vi "set Reference Level.vi"(8 "error in (no error)":errorcluster, 10 "Reference Level":dbl, 11 "Keysight 9020A in":refnum<class "Keysight 9020A.lvclass">) -> (0 "error out":errorcluster, 3 "Keysight 9020A out":refnum<class "Keysight 9020A.lvclass">)   [LabVIEW 2023, in "Spectrum Analyzer.lvlib" / "Keysight 9020A.lvclass"]
uses:
  Keysight 9020A.lvclass
  Keysight 9020A.lvclass/Keysight 9020A.ctl
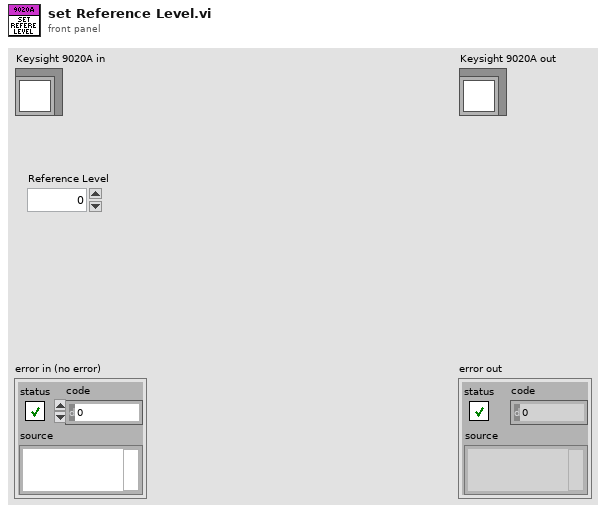
[diagram p1: front panel]
types:
  T1 = typedef "Spectrum Analyzer.lvlib/TYPE Measurement Preset.ctl" = enum16{"Sweep SA Mode", "Channel Power", "Occupied BW", "ACP", "Spurious Emission", "Spurious Emission Mask", "Burst Power (Transmit Power)"}
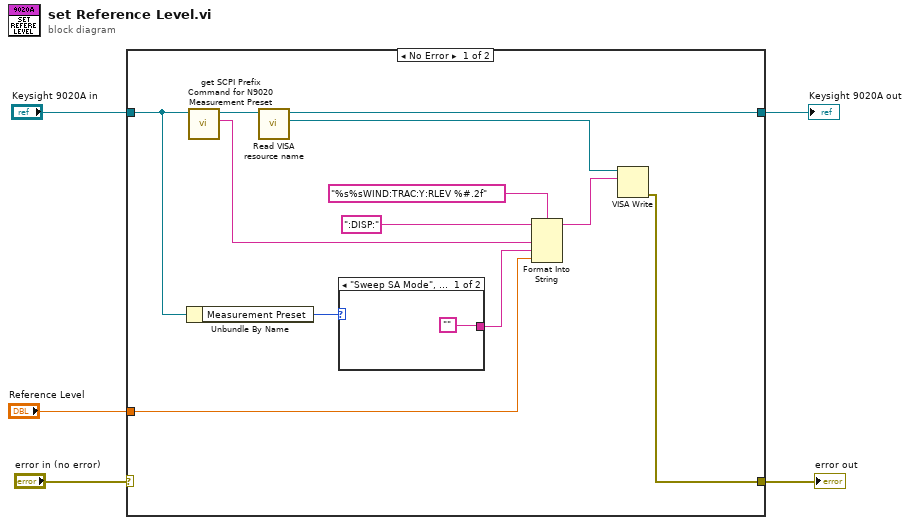
[diagram p0: block diagram]
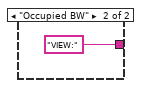
[diagram p2: hidden frame]
diagram:
  n1 = case shown="No Error" "error in (no error)" {
    selector: "error in (no error)" -> [_ w20]
    tunnel: "Keysight 9020A in" -> [w8 w21]
    tunnel: [w17 w21] -> w4
    tunnel: [w12 w20] -> w2
    tunnel: "Reference Level" -> [w6 _]
    frame No Error {
      n2 = Unbundle By Name(w8) -> ("Measurement Preset"=w9:T1)
      n3 = call "get SCPI Prefix Command for N9020 Measurement Preset.vi"("Keysight 9020A in"=w8) -> ("SCPI Prefix Command"=w10:string, "Keysight 9020A out"=w11:refnum<class "Keysight 9020A.lvclass">)  [unwired: 8 in, 1 out]
      n4 = call "Read VISA resource name.vi"("Keysight 9020A in"=w11) -> ("VISA resource name"=w14:refnum<visa-resource-name>, "Keysight 9020A out"=w17:refnum<class "Keysight 9020A.lvclass">)  [unwired: 8 in, 1 out]
      n5 = case shown="\"Sweep SA Mode\", Default" w9 {
        tunnel: ["" "VIEW:"] -> w7
        frame "Sweep SA Mode", Default {
        }
        frame "Occupied BW" {
        }
      }
      n6 = Format Into String(format string="%s%sWIND:TRAC:Y:RLEV %#.2f", initial string=":DISP:", w10, w7, w6) -> (resulting string=w13:string)  [unwired: 1 in, 1 out]
      n7 = VISA Write(VISA resource name=w14, write buffer=w13) -> (error out=w12:errorcluster)  [unwired: 1 in, 2 out]
    }
    frame Error {
    }
  }
  "error out" <- w2
  "Keysight 9020A out" <- w4
